vi "GDSLvClass_GetClassInfo.vi"(0 "Class Refnum In":refnum<vi>, 5 "error in (no error)":errorcluster) -> (14 "Class Refnum Out":refnum<vi>, 15 "ClassCtl-file":string, 16 "ClassInfo":T1, 17 "ClassMemberPath":path, 18 "Is Interface":bool, 19 "error out":errorcluster)   [LabVIEW 2020]
uses:
  GDSLvClass_ClassInfo.ctl
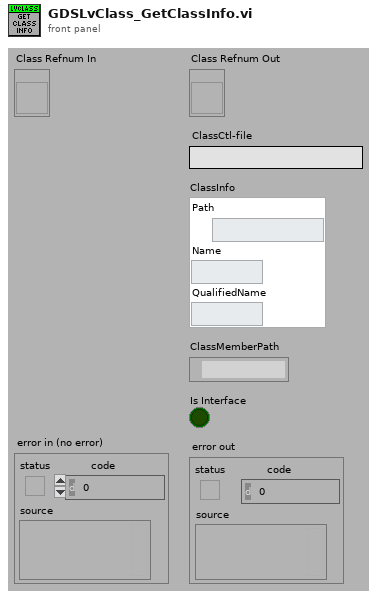
[diagram p1: front panel]
types:
  T1 = typedef "GDSLvClass_ClassInfo.ctl" = cluster{"Path":path, "Name":string, "QualifiedName":string}
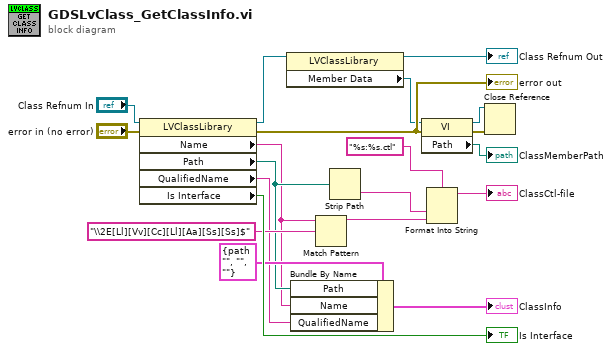
[diagram p0: block diagram]
diagram:
  n1 = property class="LVClassLibrary"(reference="Class Refnum In", error in="error in (no error)") -> (reference out=w8:refnum<vi>, error out=w19:errorcluster, "Name"=w2:string, "Path"=w3:path, "QualifiedName"=w1:string, "Is Interface"=→"Is Interface":bool)
  "error out" <- w19
  n2 = property class="LVClassLibrary"(reference=w8) -> (reference out=→"Class Refnum Out":refnum<vi>, "Member Data"=w7:refnum<vi>)  [unwired: 1 in, 1 out]
  n3 = Bundle By Name(cluster=T1 {"Path"=path "", "Name"="", "QualifiedName"=""} ("ClassInfo"), "Path"=w3, "Name"=w2, "QualifiedName"=w1) -> (→"ClassInfo":T1)
  n4 = Match Pattern(string=w2, regular expression="\\2E[Ll][Vv][Cc][Ll][Aa][Ss][Ss]$") -> (before substring=w9:string)  [unwired: 1 in, 3 out]
  n5 = Strip Path(path=w3) -> (name=w12:string)  [unwired: 1 out]
  n6 = property class="VI"(reference=w7, error in=w19) -> (reference out=w5:refnum<vi>, error out=w6:errorcluster, "Path"=→"ClassMemberPath":path)
  n7 = Format Into String(format string="%s:%s.ctl", w12, w9) -> (resulting string=→"ClassCtl-file":string)  [unwired: 2 in, 1 out]
  n8 = Close Reference(reference=w5, error in (no error)=w6) -> ()  [unwired: 1 out]
